vi "thermal_optical_capture_8.vi"() -> ()   [LabVIEW 2025]
panel:
  in  "Stop Acquisition":bool
  out "File Name Out":string
  in  "File Path":string="C:\\Digambar\\Metal_thin_wall\\Optical_images\\Optical_images"
  out "Optical Preview":T1(plugin-control)
  in  "Focus":dbl(slide) scale=0.0..100.0
  out "Thermal Frame Out":string
  in  "Thermal Output Folder":path
  in  "thermal capture interval (s)":dbl
  in  "Flag Button":bool
  in  "Stop & Save":bool
  in  "Record":bool
  # "(1) Run VI"
  # "(2) After thermal camera calibration message (in terminal), press START"
  # "(3) Stop & Save"
  # "THERMAL CONTROLS"
  # "(Enter \"28\")"
  # "Thermal Record"
  # "OPTICAL CONTROLS"
  # "(must be an empty folder)"
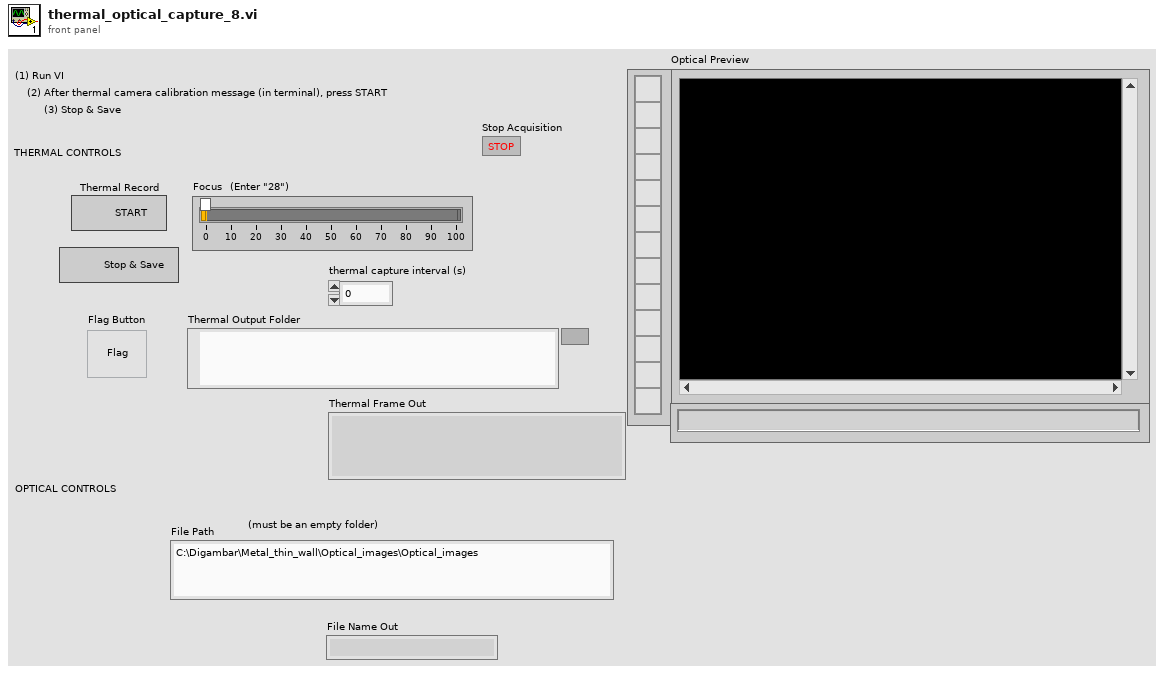
[diagram p1: front panel]
types:
  T1 = typedef "IMAQ Image.ctl" = refnum<image>
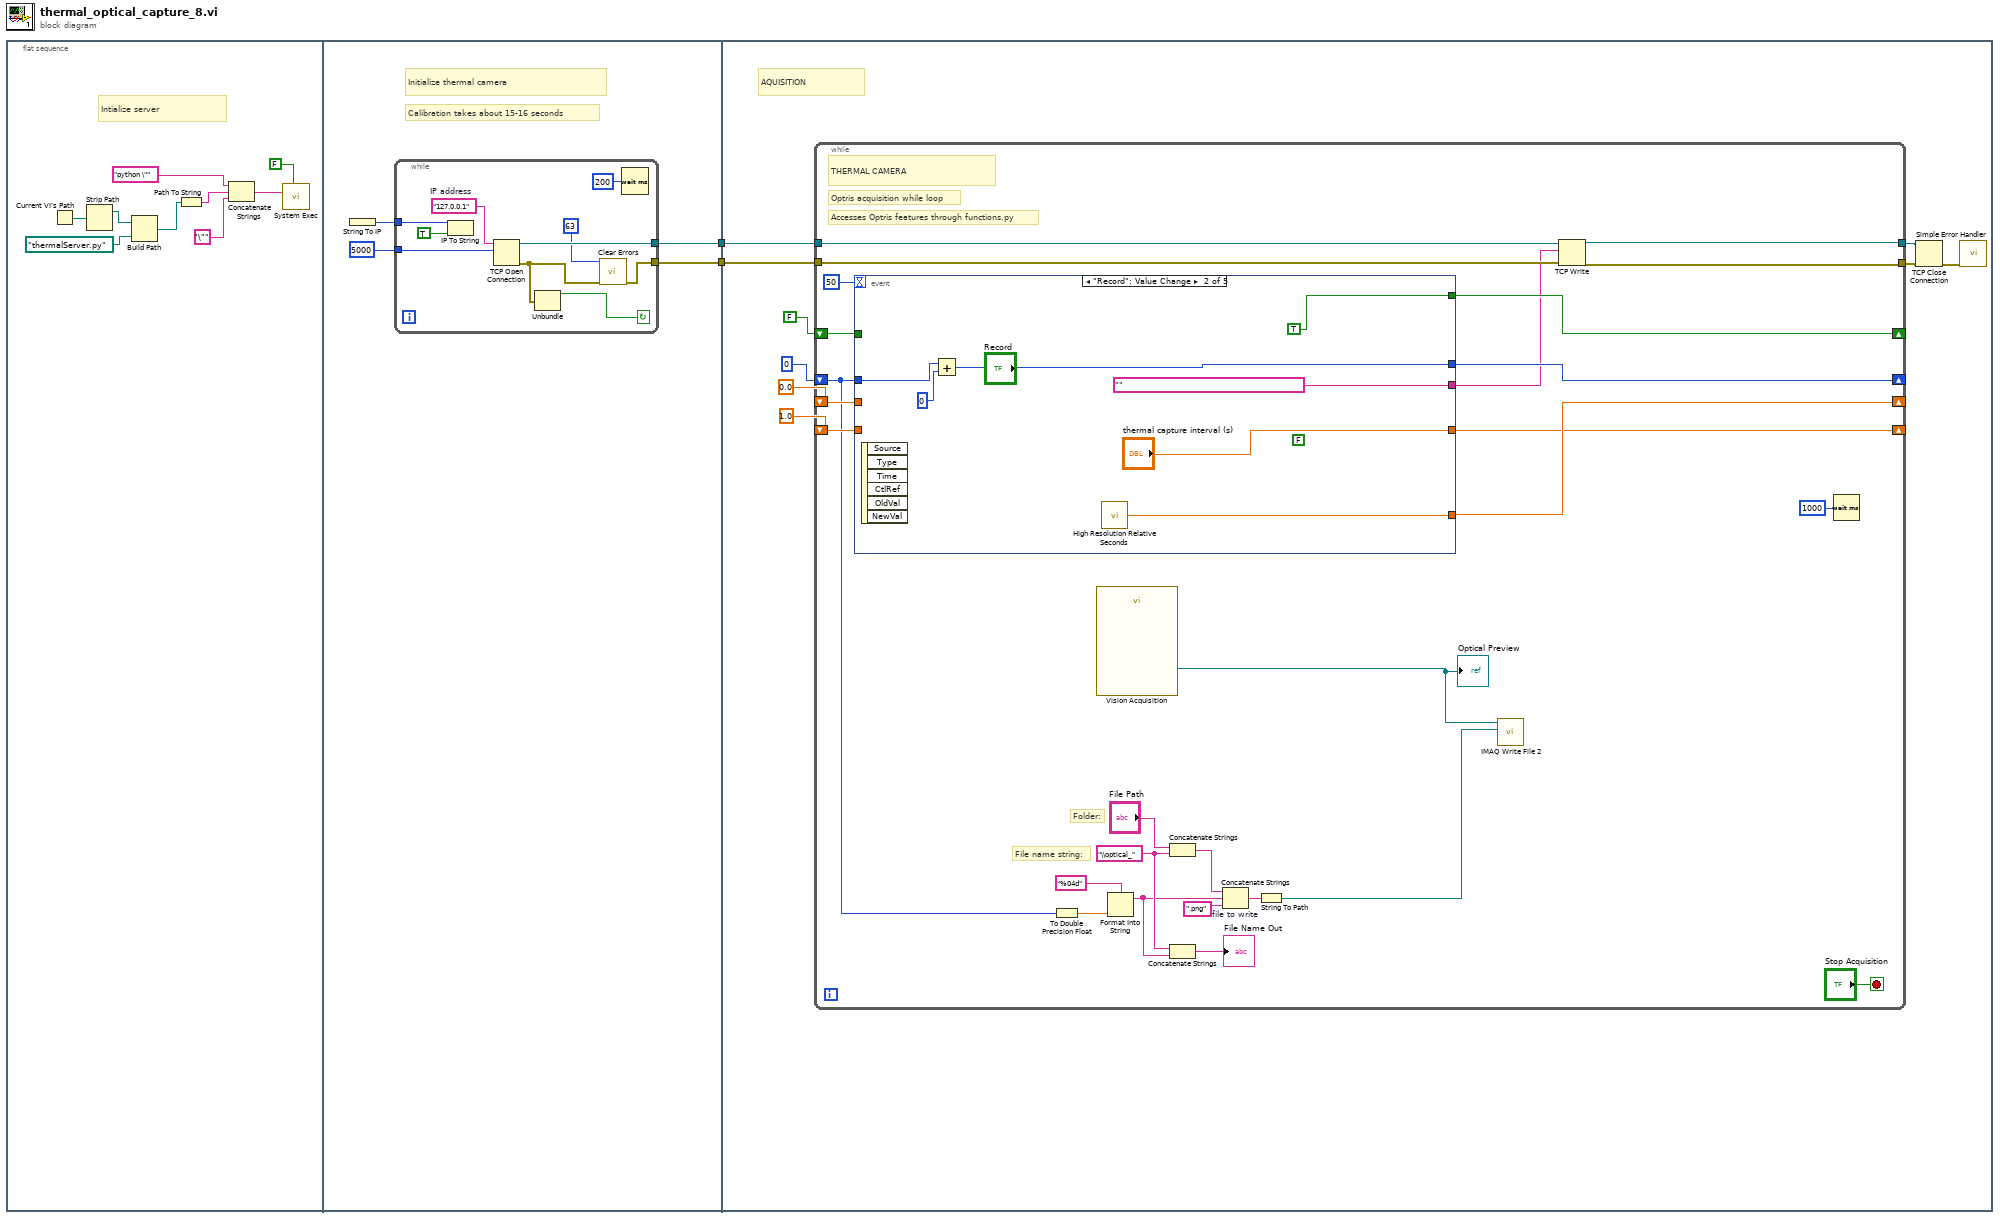
[diagram p0: block diagram]
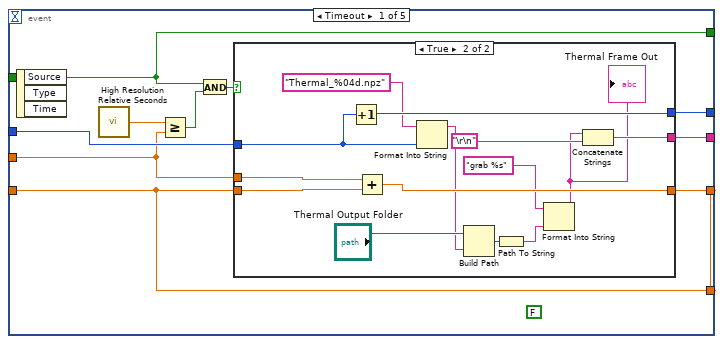
[diagram p2: hidden frame]
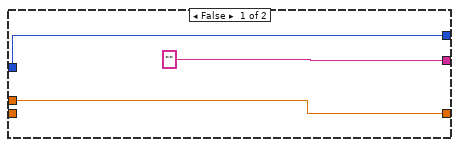
[diagram p3: hidden frame]
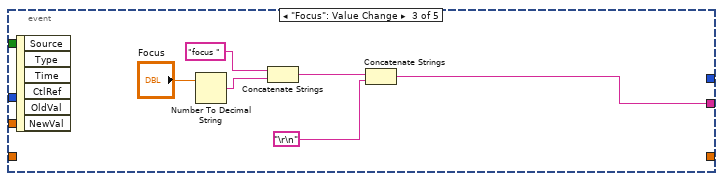
[diagram p4: hidden frame]
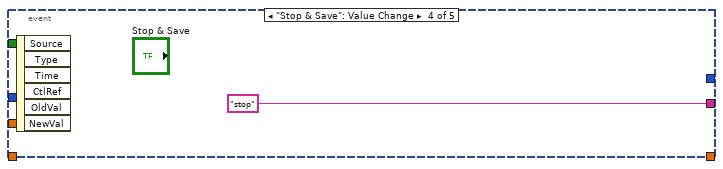
[diagram p5: hidden frame]
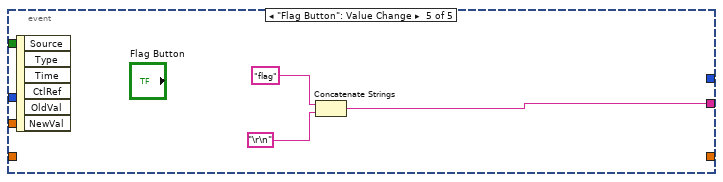
[diagram p6: hidden frame]
diagram:
  n1 = flat-sequence {
    tunnel: [w13] -> w2
    tunnel: [w12] -> w1
    tunnel: w1 -> [w31]
    tunnel: w2 -> [w30]
    frame #0 {
      # "Intialize server"
      n2 = Current VI's Path() -> (path=w6:path)
      n3 = Strip Path(path=w6) -> (stripped path=w7:path)  [unwired: 1 out]
      n4 = Build Path(base path=w7, name or relative path=path "thermalServer.py") -> (appended path=w4:path)
      n5 = Path To String(path=w4) -> (string=w10:string)
      n6 = Concatenate Strings("python \"" ("string"), w10, "\"" ("string")) -> (w9:string)
      n7 = call <vilib>:"System Exec.vi"("wait until completion? (T)"=FALSE, "command line"=w9) -> ()  [unwired: 6 in, 4 out]
    }
    frame #1 {
      # "Initialize thermal camera"
      # "Calibration takes about 15-16 seconds"
      n8 = String To IP() -> (0:w15:u32)  [unwired: 1 in]
      n9 = while {
        tunnel: [w20] -> w13
        tunnel: [w25] -> w12
        tunnel: w15 -> [w24]
        tunnel: u16 5000 ("remote port or service name") -> [w22]
        stop <- w17 continue-if-true
        w16 = "127.0.0.1"  # IP address
        n10 = IP To String(1:TRUE ("dot notation? (F)"), 2:w24) -> ()  [unwired: 1 out]
        n11 = TCP Open Connection(address=w16, remote port or service name=w22) -> (connection ID=w25:refnum<k5>, error out=w21:errorcluster)  [unwired: 3 in]
        n12 = Unbundle(w21) -> ("status"=w17:bool)  [unwired: 2 out]
        n13 = call <vilib>:"Clear Errors.vi"("error in (no error)"=w21, "specific error code to clear (0: all)"=63) -> ("error out"=w20:errorcluster)  [unwired: 4 in, 1 out]
        n14 = Wait (ms)(milliseconds to wait=u32 200) -> ()  [unwired: 1 out]
      }
    }
    frame #2 {
      # "AQUISITION"
      n15 = while {
        tunnel: [w61] -> w32
        tunnel: [w60] -> w33
        tunnel: w31 -> [w59]
        tunnel: w30 -> [w58]
        shift-right: [w57] -> _
        shift-left: u32 0 -> [w36]
        shift-right: [w56] -> _
        shift-left: 0.0 -> [w52]
        shift-right: [w53] -> _
        shift-left: 1.0 -> [w50]
        shift-right: [w54] -> _
        shift-left: FALSE -> [w51]
        stop <- "Stop Acquisition" stop-if-true
        w43 = "\\optical_" ("string")
        # "Folder:"
        # "File name string:"
        # "THERMAL CAMERA"
        # "Optris acquisition while loop"
        # "Accesses Optris features through functions.py"
        n16 = event shown="[1] \"Record\": Value Change" {
          selector: _ -> [_ _ _ _ _]
          dyn-events: _ -> [_ _ _ _ _]
          timeout: 50 -> [_ _ _ _ _]
          tunnel: [w67 "" w96 "stop" w105] -> w49
          tunnel: w36 -> [w68 w95 _ _ _]
          tunnel: [w66 w93 _ _ _] -> w57
          tunnel: [w64 w92 _ _ _] -> w56
          tunnel: [w62 TRUE _ _ _] -> w54
          tunnel: [w63 "thermal capture interval (s)" _ _ _] -> w53
          tunnel: w52 -> [w65 _ _ _ _]
          tunnel: w51 -> [w62 _ _ _ _]
          tunnel: w50 -> [w63 _ _ _ _]
          event Timeout {
            (unwired) FALSE
            n17 = event-data() -> ()  [unwired: 1 in, 3 out]
            n18 = call <vilib>:"High Resolution Relative Seconds.vi"() -> ("relative seconds"=w71:dbl)
            n19 = Greater Or Equal?(x=w71, y=w65) -> (x >= y?=w70:bool)
            n20 = And(x=w62, y=w70) -> (x .and. y?=w69:bool)
            n21 = case shown="True" w69 {
              tunnel: w68 -> [w73 w86]
              tunnel: ["" w87] -> w67
              tunnel: [w73 w85] -> w66
              tunnel: w65 -> [w72 w84]
              tunnel: w63 -> [_ w83]
              tunnel: [w72 w82] -> w64
              frame False {
              }
              frame True {
                n22 = Increment(x=w86) -> (x+1=w85:u32)
                n23 = Add(x=w84, y=w83) -> (x+y=w82:dbl)
                n24 = Format Into String(format string="Thermal_%04d.npz", w86) -> (resulting string=w77:string)  [unwired: 2 in, 1 out]
                n25 = Build Path(base path="Thermal Output Folder", name or relative path=w77) -> (appended path=w79:path)
                n26 = Path To String(path=w79) -> (string=w76:string)
                n27 = Format Into String(format string="grab %s", w76) -> (resulting string=w75:string)  [unwired: 2 in, 1 out]
                "Thermal Frame Out" <- w75
                n28 = Concatenate Strings(w75, "\r\n") -> (w87:string)
              }
            }
          }
          event "Record": Value Change {
            (unwired) FALSE
            n29 = event-data() -> ()  [unwired: 1 in, 6 out]
            n30 = Add(x=w95, y=u32 0) -> (x+y=w93:u32)
            n31 = call <vilib>:"High Resolution Relative Seconds.vi"() -> ("relative seconds"=w92:dbl)
          }
          event "Focus": Value Change {
            n32 = event-data() -> ()  [unwired: 1 in, 6 out]
            n33 = Number To Decimal String(number="Focus") -> (decimal integer string=w101:string)  [unwired: 1 in]
            n34 = Concatenate Strings("focus ", w101) -> (w98:string)
            n35 = Concatenate Strings(w98, "\r\n") -> (w96:string)
          }
          event "Stop & Save": Value Change {
            n36 = event-data() -> ()  [unwired: 1 in, 6 out]
          }
          event "Flag Button": Value Change {
            n37 = event-data() -> ()  [unwired: 1 in, 6 out]
            n38 = Concatenate Strings("flag", "\r\n") -> (w105:string)
          }
        }
        n39 = To Double Precision Float(number=w36) -> (double precision float=w41:dbl)
        n40 = call "Vision Acquisition"() -> ("Image Out"=w48:T1)  [unwired: 26 in, 1 out]
        "Optical Preview" <- w48
        n41 = Format Into String(format string="%04d" ("time format string (%c)"), w41) -> (resulting string=w39:string)  [unwired: 2 in, 1 out]
        n42 = Concatenate Strings("File Path", w43) -> (w44:string)
        n43 = Concatenate Strings(w43, w39) -> (→"File Name Out":string)
        n44 = Concatenate Strings "file to write"(w44, w39, ".png" ("string")) -> (w47:string)
        n45 = String To Path(string=w47) -> (path=w40:path)
        n46 = call-poly "IMAQ Write File 2"("File Path"=w40, "Image"=w48) -> ()  [unwired: 8 in, 2 out]
        n47 = TCP Write(connection ID=w59, data in=w49, error in (no error)=w58) -> (connection ID out=w60:refnum<k5>, error out=w61:errorcluster)  [unwired: 1 in, 1 out]
        n48 = Wait (ms)(milliseconds to wait=u32 1000) -> ()  [unwired: 1 out]
      }
      n49 = TCP Close Connection(connection ID=w33, error in (no error)=w32) -> (error out=w34:errorcluster)  [unwired: 1 in, 1 out]
      n50 = call <vilib>:"Simple Error Handler.vi"("error in (no error)"=w34) -> ()  [unwired: 4 in, 5 out]
    }
  }
